vi "Read I16.vi"(8 "error in (no error)":errorcluster, 11 "Event in":refnum<class "Event I16.lvclass">) -> (0 "error out":errorcluster, 2 "I16":i16, 3 "Event out":refnum<class "Event I16.lvclass">)   [LabVIEW 2023, in "MVC Actors.lvlib" / "Event I16.lvclass"]
uses:
  Event I16.lvclass
  Event I16.lvclass/Event I16.ctl
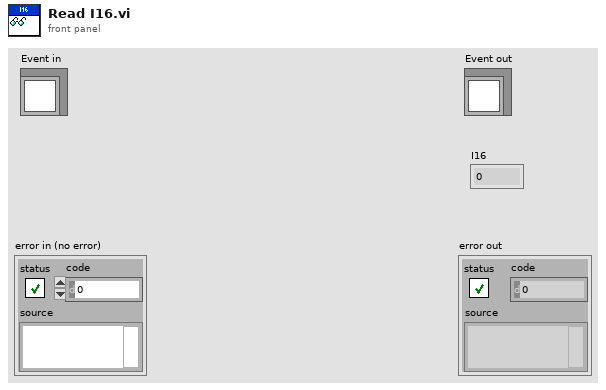
[diagram p1: front panel]
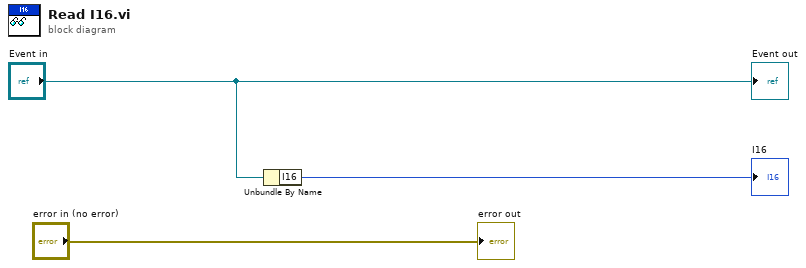
[diagram p0: block diagram]
diagram:
  n1 = Unbundle By Name("Event in") -> ("I16"=→"I16":i16)
  "Event out" <- "Event in"
  "error out" <- "error in (no error)"
